vi "Host_State_Update.vi"(8 "error in (no error)":errorcluster={"status"=FALSE, "code"=0, "source"="\"\""}, 10 "existing Host state":string, 11 "Incoming runtime event":string) -> (0 "error out":errorcluster={"status"=FALSE, "code"=0, "source"="\"\""}, 2 "status ok":bool, 3 "New Host state":string)   [LabVIEW 2026]
doc: "INTENT: Build consistent HMI view model. LOGIC: Match run ID and event sequence; update status, active step, progress and operator notices."
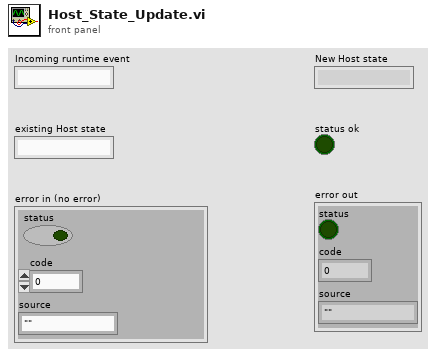
[diagram p1: front panel]
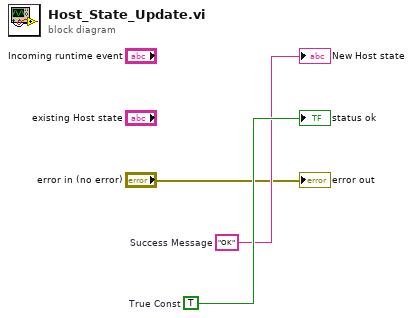
[diagram p0: block diagram]
diagram:
  w3 = TRUE  # True Const
  w2 = "OK"  # Success Message
  "New Host state" <- w2
  "status ok" <- w3
  "error out" <- "error in (no error)"
